vi "FPGA.vi"() -> ()   [LabVIEW 2025]
uses:
  Cluster_TH.ctl
  <vilib>/rvi/Emulation/niFpgaGetClockAttributes.vi
  <vilib>/rvi/Emulation/niFpgaSctlEmulationGetInTimedLoop.vi
  <vilib>/rvi/Emulation/niFpgaEmulationReportErrorSimple.vi
  <vilib>/rvi/Emulation/niFpgaEmulationIsFPGAContextNoSignature.vi
  <vilib>/rvi/errors/niFpgaSetErrorForExecOnDevCompSimple.vi
  <vilib>/rvi/eio/common/nirviEmuReportErrorAndStop.vi
  <vilib>/rvi/DataTransferAndStorage/Container/Common/niFpgaContainerGetUniqueNameForEmu.vi
  <vilib>/rvi/FIFO/Fifo_Resource/nirvififoEmulationSetSize.vi
  <vilib>/rvi/FIFO/Fifo_Resource/nirviFifoEmulationQueueMgr.vi
  <instcachedir>/0/nirviFifoEmulationQueueMgr_E5CAEC123FF24DC58D834DCA3CDAA9B5.lvgen/nirviFifoEmulationQueueMgr_E5CAEC123FF24DC58D834DCA3CDAA9B5_001.vi
  <vilib>/Utility/error.llb/Clear Errors.vi
  <vilib>/rvi/FIFO/Fifo_Resource/nirvififoEmulationCreateLock.vi
  <vilib>/rvi/Emulation/niFpgaProcessEmulError.vi
  <vilib>/rvi/FIFO/Fifo_Resource/nirvififoEmulationObtainLock.vi
  <vilib>/rvi/FIFO/Fifo_Resource/nirvififoEmulationReleaseLock.vi
  <vilib>/rvi/occurrence/nirviWaitOnOccurrenceBase.vi
  <vilib>/rvi/errors/nirviReportUnexpectedCaseInternalError.vi
  <vilib>/rvi/errors/nirviReportUnexpectedCaseInternalError (U32).vi
  <vilib>/eio/utilities/niEioResolveVilibRelativePath.vi
  <vilib>/rvi/interface/RandomDataEmulation/niFpgaRandomDataHandleErrors.vi
  <vilib>/rvi/Emulation/niFpgaCriticalErrorInLSC.vi
  <vilib>/rvi/eio/common/nirviEmuTemplateMethod_errors.vi
  <vilib>/rvi/Memory/Memory_Emulation/nirvimemoryFastEmulation.vi
  <vilib>/rvi/Memory/Memory_Emulation/nirvimemoryEmulation.vi
  <vilib>/rvi/DataTransferAndStorage/Container/Common/niFpgaContainerExecOnDevCompGetState.vi
  <vilib>/rvi/Memory/Memory_Emulation/niFpgaMemoryEmulationCacheClearOnFirstRun.vi
  <vilib>/rvi/Memory/Memory_Emulation/nirvimemoryEmulationManagerCache_MakeExclusive.vi
  <vilib>/rvi/Memory/Memory_Emulation/niFpgaMemoryEmulationValidateCache.vi
  <vilib>/rvi/Memory/Memory_Emulation/nirvimemoryEmulationManagerCache_InsertValue.vi
  <vilib>/rvi/Memory/Memory_Emulation/nirvimemoryEmulationManagerCache_ReleaseExclusive.vi
  <vilib>/rvi/Memory/Memory_Emulation/nirvimemoryEmulationManagerCache_GetValue.vi
  <vilib>/rvi/Memory/Memory_Emulation/nirvimemoryEmulationManagerCache_SetValue.vi
  <vilib>/rvi/Emulation/niFpgaSctlEmulationResourceMgr.vi
  <vilib>/rvi/FIFO/Fifo_Resource/nirvififoEmulationDetermineInputValidOut.vi
  <vilib>/rvi/DataTransferAndStorage/Container/XNode/niFpgaContainer.xnode
  <vilib>/rvi/FIFO/Fifo_Resource/nirvififoEmulationRead.vi
  <vilib>/rvi/interface/RandomDataEmulation/nirviRandomDataFpgaReadWriteTemplate.vi
  <vilib>/eio/EIONode/EIONode.xnode
  <vilib>/rvi/Memory/Memory_Emulation/niFpgaMemoryEmulationRefIn.vi
  <vilib>/rvi/FIFO/Fifo_Resource/nirvififoEmulationWrite.vi
panel:
  in  "THs":T1={"X_TH"=400, "Y_TH"=400, "Z_TH"=400}
  in  "Count(uSec)":u32=1250
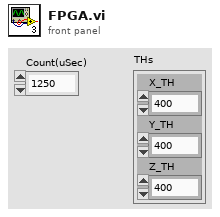
[diagram p1: front panel]
types:
  T1 = typedef "Cluster_TH.ctl" = cluster{"X_TH":i16, "Y_TH":i16, "Z_TH":i16}
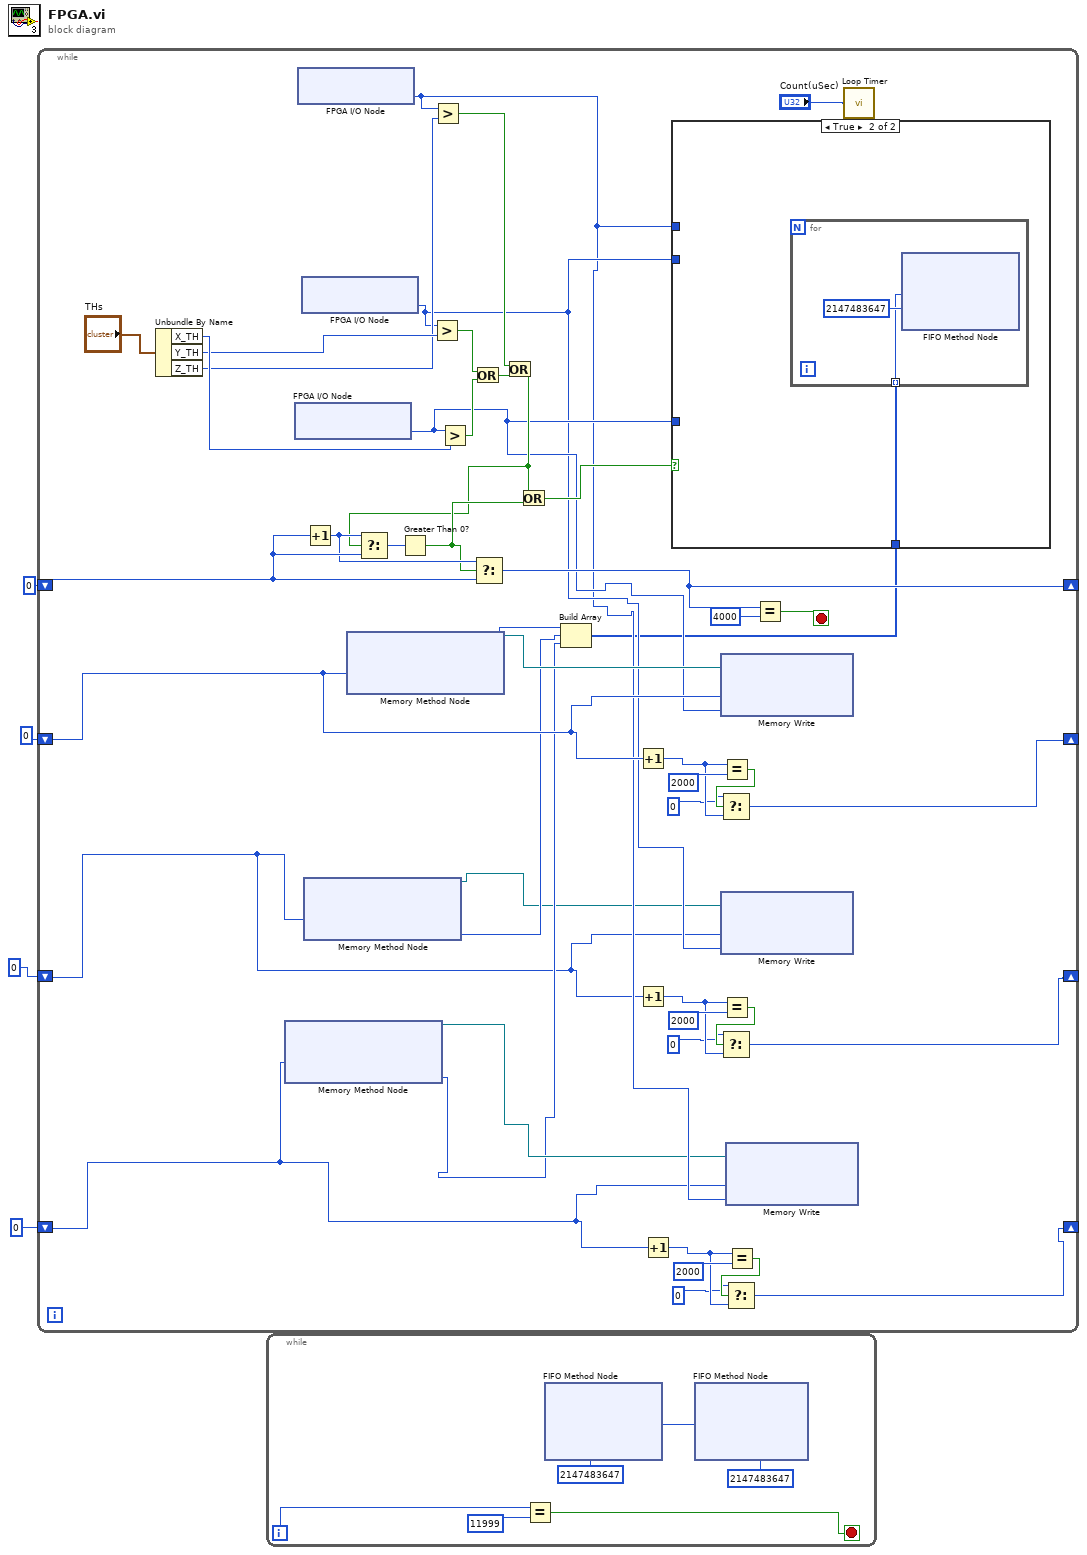
[diagram p0: block diagram]
diagram:
  n1 = while {
    shift-right: [w43] -> _
    shift-left: 0 ("y") -> [w47]
    shift-right: [w29] -> _
    shift-left: u32 0 ("t") -> [w31]
    shift-right: [w16] -> _
    shift-left: u32 0 ("t") -> [w7]
    shift-right: [w15] -> _
    shift-left: u32 0 ("t") -> [w8]
    stop <- w49 stop-if-true
    n2 = Unbundle By Name("THs") -> ("X_TH"=w40:i16, "Y_TH"=w39:i16, "Z_TH"=w38:i16)
    n3 = xnode ("Memory Method Node")("Address"=w8) -> ("Data"=w9:i16, "Memory Out"=w10:refnum<k21>)  [unwired: 1 in]
    n4 = xnode "FPGA I/O Node"() -> ("AccelerationX"=w25:i16)  [unwired: 1 in, 1 out]
    n5 = xnode "FPGA I/O Node"() -> ("AccelerationZ"=w13:i16)  [unwired: 1 in, 1 out]
    n6 = xnode "FPGA I/O Node"() -> ("AccelerationY"=w14:i16)  [unwired: 1 in, 1 out]
    n7 = xnode ("Memory Method Node")("Address"=w7) -> ("Data"=w6:i16, "Memory Out"=w5:refnum<k21>)  [unwired: 1 in]
    n8 = Increment(x=w47) -> (x+1=w46:i32)
    n9 = xnode ("Memory Method Node")("Address"=w31) -> ("Data"=w12:i16, "Memory Out"=w32:refnum<k21>)  [unwired: 1 in]
    n10 = Greater?(x=w14, y=w39) -> (0:w35:bool)
    n11 = Greater?(x=w13, y=w38) -> (0:w36:bool)
    n12 = Greater?(x=w25, y=w40) -> (0:w34:bool)
    n13 = Or(x=w35, y=w34) -> (x .or. y?=w37:bool)
    n14 = Or(x=w36, y=w37) -> (x .or. y?=w33:bool)
    n15 = Select(t=w46, s=w33, f=w47) -> (s? t:f=w48:i32)
    n16 = Greater Than 0?(x=w48) -> (x > 0?=w45:bool)
    n17 = Select(t=w46, s=w45, f=w47) -> (s? t:f=w43:i32)
    n18 = Or(x=w33, y=w45) -> (x .or. y?=w42:bool)
    n19 = Build Array(w12, w6, w9) -> (w11:i16[])
    n20 = Increment(x=w31) -> (x+1=w27:u32)
    n21 = Increment(x=w7) -> (x+1=w22:u32)
    n22 = Increment(x=w8) -> (x+1=w18:u32)
    n23 = case shown="True" w42 {
      tunnel: w25 -> [_ _]
      tunnel: w14 -> [_ _]
      tunnel: w13 -> [_ _]
      tunnel: w11 -> [_ w51]
      frame False {
      }
      frame True {
        n24 = for {
          tunnel: w51 -> [w52] mode=indexing
          n25 = xnode ("FIFO Method Node")("Element"=w52, "Timeout"=2147483647) -> ()  [unwired: 1 in, 2 out]
        }
      }
    }
    n26 = xnode ("Memory Write")("Address"=w31, "Data"=w25, "Memory In"=w32) -> ()  [unwired: 1 out]
    n27 = xnode ("Memory Write")("Address"=w7, "Data"=w14, "Memory In"=w5) -> ()  [unwired: 1 out]
    n28 = Equal?(x=w27, y=u32 2000) -> (x = y?=w30:bool)
    n29 = Select(t=u32 0, s=w30, f=w27) -> (s? t:f=w29:u32)
    n30 = Equal?(x=w22, y=u32 2000) -> (x = y?=w24:bool)
    n31 = Select(t=u32 0, s=w24, f=w22) -> (s? t:f=w16:u32)
    n32 = xnode ("Memory Write")("Address"=w8, "Data"=w13, "Memory In"=w10) -> ()  [unwired: 1 out]
    n33 = Equal?(x=w18, y=u32 2000) -> (x = y?=w20:bool)
    n34 = Select(t=u32 0, s=w20, f=w18) -> (s? t:f=w15:u32)
    n35 = Equal?(x=w43, y=4000) -> (x = y?=w49:bool)
    n36 = call "Loop Timer"("Count(uSec)"="Count(uSec)") -> ()  [unwired: 1 out]
  }
  n37 = while {
    i -> [w56]
    stop <- w54 stop-if-true
    n38 = Equal?(x=w56, y=11999) -> (x = y?=w54:bool)
    n39 = xnode ("FIFO Method Node")("Timeout"=2147483647) -> ("Element"=w58:i16)  [unwired: 1 in, 2 out]
    n40 = xnode ("FIFO Method Node")("Element"=w58, "Timeout"=2147483647) -> ()  [unwired: 1 in, 2 out]
  }
